vi "报警.vi"() -> ()   [LabVIEW 2026]
doc: "报警规则设置界面 - APS 测控软件 飞机辅助动力装置。仅前面板布局演示，无程序逻辑。来源：报警.html 主界面。"
panel:
  out "16 状态栏-操作提示":string="操作提示：勾选左侧「启用」列可开关单条规则 · 修改阈值即时生效"
  out "15 状态栏-触发次数":string="触发次数: 4"
  out "14 状态栏-启用规则":string="启用规则: 22"
  out "13 状态栏-规则状态":string="规则状态: 正常"
  out "12 实时信号监测":string[](array[string])=["转速[下位机TCP] 27540 rpm", "排气温度[下位机TCP] 645 ℃", "滑油压力[下位机TCP] 348 kPa", "燃油流量[下位机TCP] 1240 kg/h", "28V母线电压[PLC OPC] 28.10 V", "发电机频率[CAN总线] 398 Hz", "气压高度[ARINC429] 3200 m"]
  out "11 统计-今日触发":string="今日触发: 0 次 · 累计: 0 次"
  out "10 统计-提示":i32
  out "09 统计-警告":i32=10
  out "08 统计-严重":i32=8
  out "07 统计-紧急":i32=2
  out "06 表格说明":string="启用规则: 22 / 25 · 模拟量按「大于/小于」阈值触发 · 开关量按「等于 0 / 等于 1」触发"
  out "05 报警规则表":string[][](array[string])=[["启用 信号名称 类型 报警条件 阈值 报警等级 操作"], ["R001 转速[下位机TCP] 模拟量 大于 30000 rpm 紧急 删除"], ["R002 转速[下位机TCP] 模拟量 小于 1200 rpm 警告 删除"], ["R003 排气温度[下位机TCP] 模拟量 大于 750 ℃ 紧急 删除"], ["R004 滑油压力[下位机TCP] 模拟量 小于 250 kPa 紧急 删除"], ["R005 滑油温度[下位机TCP] 模拟量 大于 130 ℃ 严重 删除"], ["R006 燃油流量[下位机TCP] 模拟量 大于 1450 kg/h 严重 删除"], ["R007 振动[下位机TCP] 模拟量 大于 4.5 g 紧急 删除"], ["R008 进气温度[下位机TCP] 模拟量 大于 50 ℃ 警告 删除"], ["R101 28V母线电压[PLC OPC] 模拟量 大于 30 V 严重 删除"], ["R102 28V母线电压[PLC OPC] 模拟量 小于 26 V 严重 删除"], ["R103 28V母线电流[PLC OPC] 模拟量 大于 22 A 严重 删除"], ["R104 气源压力[PLC OPC] 模拟量 小于 420 kPa 警告 删除"], ["R201 发电机频率[CAN总线] 模拟量 大于 420 Hz 严重 删除"], ["R202 发电机频率[CAN总线] 模拟量 小于 380 Hz 严重 删除"], ["R203 发电机电压[CAN总线] 模拟量 大于 270 V 严重 删除"], ["R204 负载电流[CAN总线] 模拟量 大于 85 A 警告 删除"], ["R301 气压高度[ARINC429] 模拟量 大于 4500 m 严重 删除"], ["R302 马赫数[ARINC429] 模拟量 大于 0.48 - 警告 删除"], ["R303 校准空速[ARINC429] 模拟量 小于 220 kt 警告 删除"], ["R304 大气总温[ARINC429] 模拟量 小于 -20 ℃ 警告 删除"], ["D001 起动信号[下位机TCP] 开关量 等于0 固定为0 警告 触发中"], ["D002 点火状态[下位机TCP] 开关量 等于0 固定为0 警告 触发中"], ["D101 气动阀状态[PLC OPC] 开关量 等于0 固定为0 警告 触发中"], ["D201 发电机状态[CAN总线] 开关量 等于0 固定为0 严重 触发中"], ["D301 429数据有效[ARINC429] 开关量 等于0 固定为0 严重 触发中"]]
  in  "测试全部规则":bool
  in  "恢复默认":bool
  in  "新增规则":bool
  in  "加载配置":bool
  in  "保存配置":bool
  in  "全部禁用":bool
  in  "全部启用":bool
  in  "类型筛选":i32(ring) items=["全部类型", "模拟量", "开关量"]
  in  "链路筛选":i32(ring) items=["全部链路", "下位机 TCP", "PLC OPC", "CAN 总线", "ARINC429"]
  out "04 时钟":string="--:--:--"
  out "03 启用数":string="启用: 22"
  out "02 规则数":string="规则数: 25"
  out "01 标题栏":string="● 报警规则设置 | APS 测控软件 · 飞机辅助动力装置"
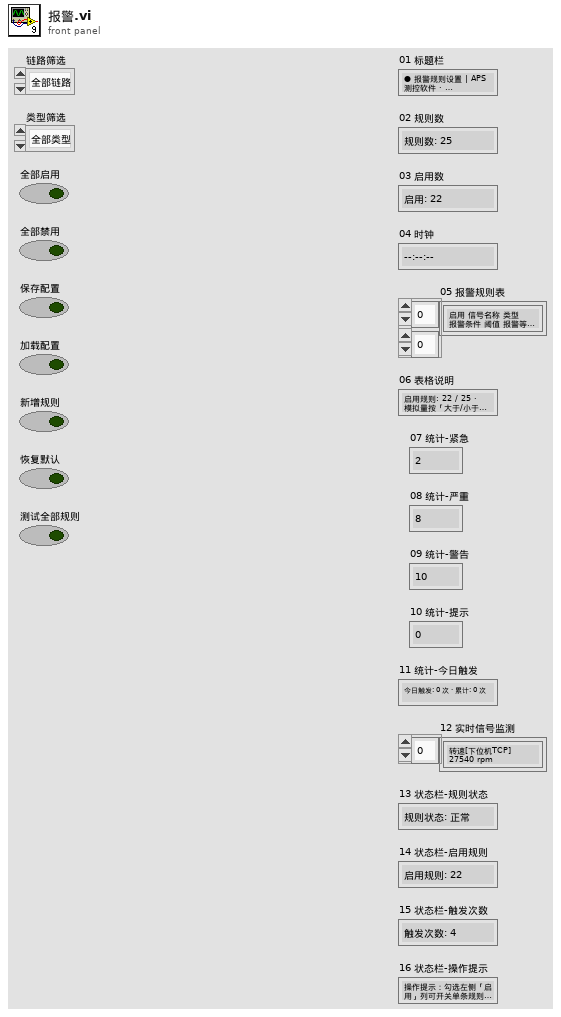
[diagram p1: front panel]
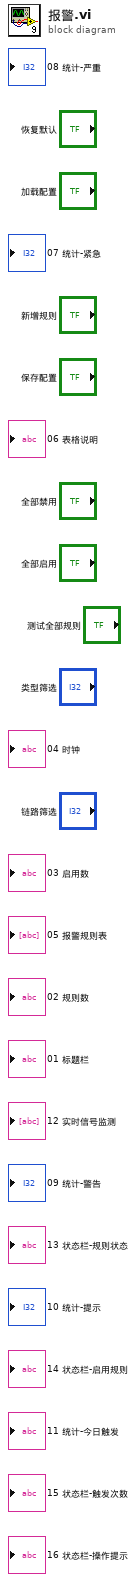
[diagram p0: block diagram]
diagram:
